vi "Read data.vi"(8 "error in (no error)":errorcluster, 11 "ZM-PC-TP-test_package in":refnum<class "ZM-PC-TP-test_package.lvclass">) -> (0 "error out":errorcluster, 2 "ZM-PC-TP-DATA":T1, 3 "ZM-PC-TP-test_package out":refnum<class "ZM-PC-TP-test_package.lvclass">)   [LabVIEW 2020, in "ZM-PC-packages.lvlib" / "ZM-PC-TP-test_package.lvclass"]
doc: "Reads one field of this class's private data. Generated by lvai_create_accessors from the class private data control."
uses:
  ZM-PC-TP-test_package.lvclass
  ZM-PC-TP-test_package.lvclass/ZM-PC-TP-test_package.ctl
  ZM-PC-TP-DATA.ctl
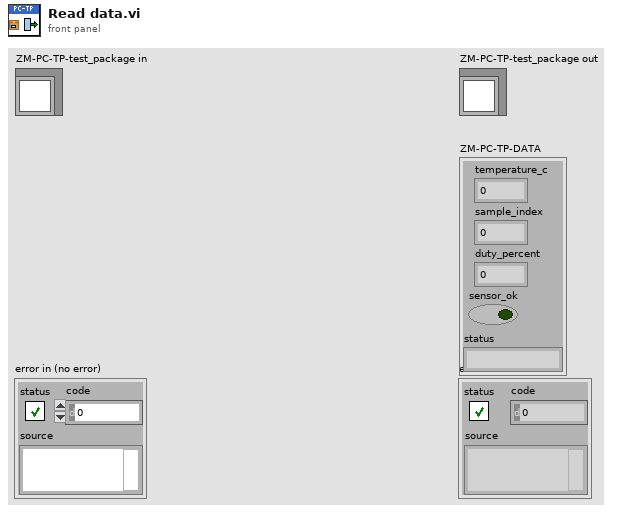
[diagram p1: front panel]
types:
  T1 = typedef "ZM-PC-packages.lvlib/ZM-PC-TP-test_package.lvclass/ZM-PC-TP-DATA.ctl" = cluster{"temperature_c":dbl, "sample_index":i32, "duty_percent":u8, "sensor_ok":bool, "status":string}
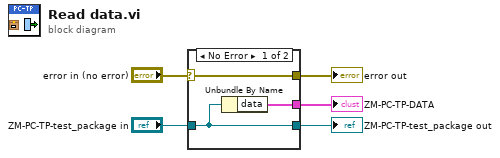
[diagram p0: block diagram]
diagram:
  n1 = case shown="No Error" "error in (no error)" {
    selector: "error in (no error)" -> [w8 w9]
    tunnel: [w8 w9] -> w4
    tunnel: [w7 w10] -> w2
    tunnel: "ZM-PC-TP-test_package in" -> [w7 w10]
    tunnel: [w6 _] -> w1
    frame No Error {
      n2 = Unbundle By Name(w7) -> ("data"=w6:T1)
    }
    frame Error {
    }
  }
  "error out" <- w4
  "ZM-PC-TP-test_package out" <- w2
  "ZM-PC-TP-DATA" <- w1
